vi "Scripting_OpenViRef.vi"(8 "error in":errorcluster, 10 "ViPath/ViName/Viref":variant, 11 "AppRef":refnum<vi>) -> (0 "error out":errorcluster, 2 "RefOpened(Needs to be closed)":bool, 3 "vi reference":refnum<vi>)   [LabVIEW 2020]
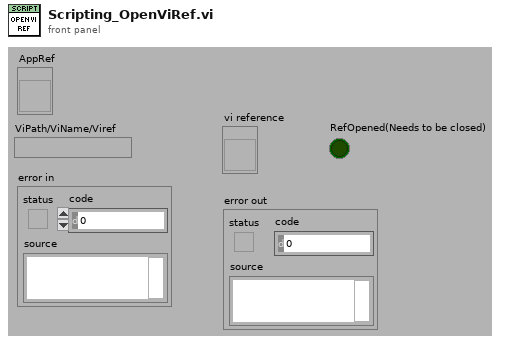
[diagram p1: front panel]
types:
  T1 = enum32{"invalid lock state", "Not Locked", "Locked (No Password)", "Password-protected"}
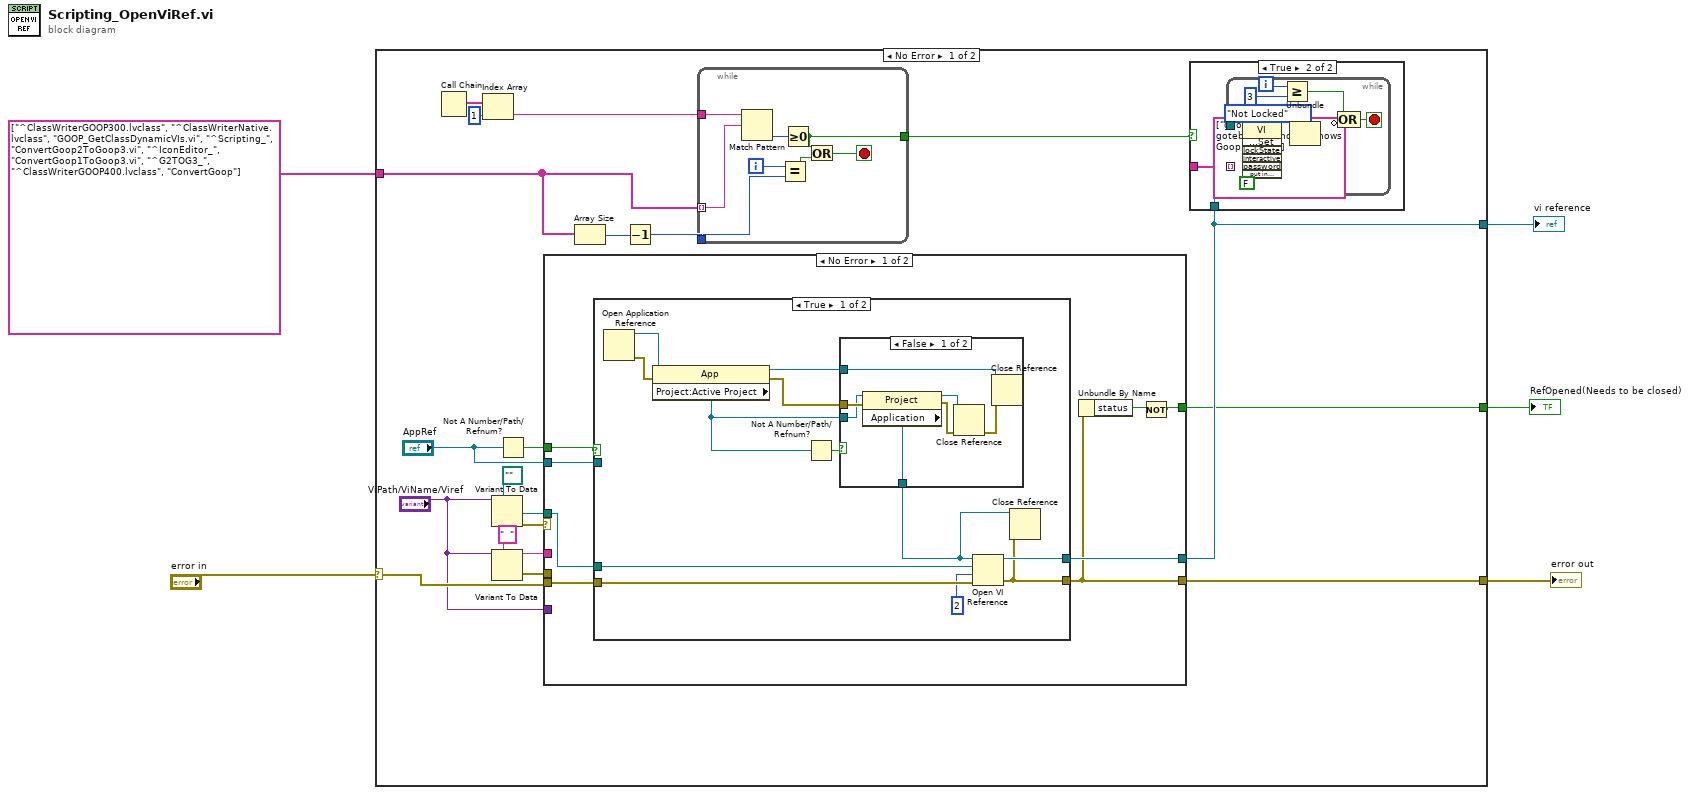
[diagram p0: block diagram]
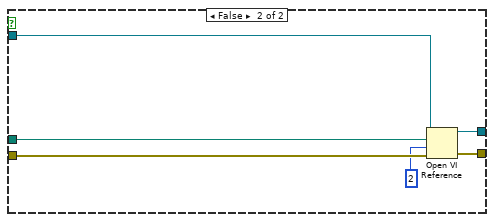
[diagram p4: hidden frame]
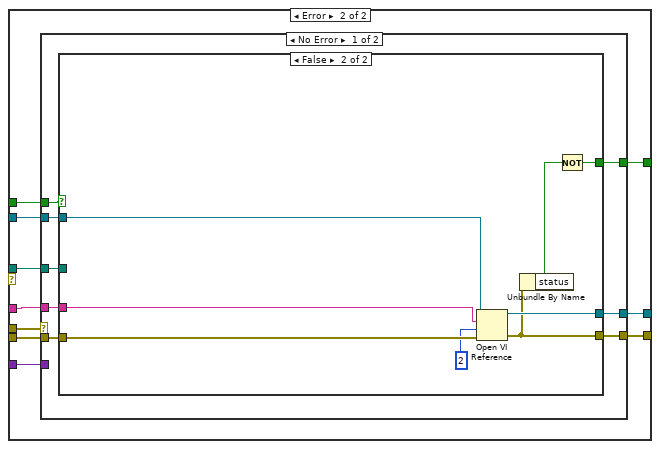
[diagram p5: hidden frame]
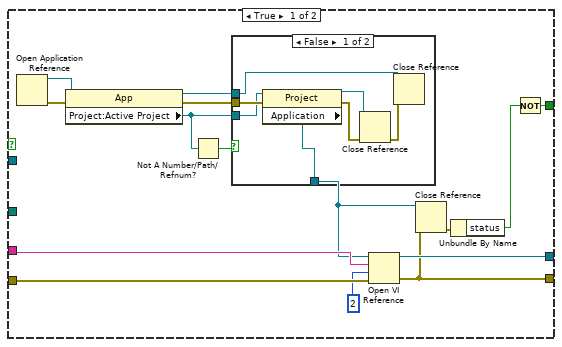
[diagram p6: hidden frame]
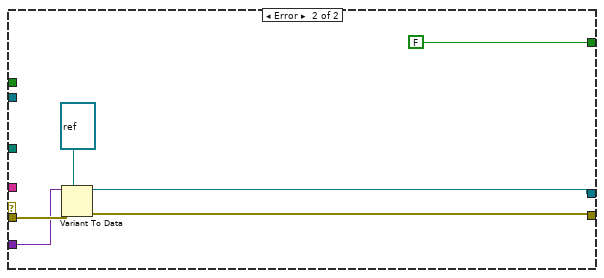
[diagram p8: hidden frame]
diagram:
  n1 = case shown="No Error" "error in" {
    selector: "error in" -> [w17 w136]
    tunnel: [w26 w136] -> w5
    tunnel: [w25 _] -> w4
    tunnel: string[] ["^ClassWriterGOOP300.lvclass", "^ClassWriterNative.lvclass", "GOOP_GetClassDynamicVIs.vi", "^Scripting_", "ConvertGoop2ToGoop3.vi", "^IconEditor_", "ConvertGoop1ToGoop3.vi", "^G2TOG3_", "^ClassWriterGOOP400.lvclass", "ConvertGoop"] -> [w9 _]
    tunnel: [w6 _] -> w1
    frame No Error {
      n2 = Call Chain() -> (call chain=w16:string[])
      n3 = Index Array(array=w16, index=1) -> (element=w14:string)
      n4 = Variant To Data(type=path "" ("vi path"), Variant="ViPath/ViName/Viref") -> (data=w23:path, error out=w22:errorcluster)  [unwired: 1 in]
      n5 = Variant To Data(type="  ", Variant="ViPath/ViName/Viref") -> (data=w18:string, error out=w8:errorcluster)  [unwired: 1 in]
      n6 = Not A Number/Path/Refnum?(number/path/refnum="AppRef") -> (NaN/Path/Refnum?=w21:bool)
      n7 = case shown="No Error" w22 {
        tunnel: w17 -> [w54 w90]
        tunnel: [w49 w89] -> w26
        tunnel: [w53 w88] -> w25
        tunnel: w23 -> [w52 w87]
        tunnel: w21 -> [w51 w86]
        tunnel: "AppRef" -> [w50 w85]
        tunnel: w18 -> [_ w84]
        tunnel: w8 -> [_ w83]
        tunnel: "ViPath/ViName/Viref" -> [_ w82]
        tunnel: [w47 w81] -> w6
        frame No Error {
          n8 = case shown="True" w51 {
            tunnel: w54 -> [w66 w80]
            tunnel: [w60 w79] -> w49
            tunnel: [w61 w78] -> w53
            tunnel: w52 -> [w64 w76]
            tunnel: w50 -> [_ w75]
            frame True {
              n9 = Open Application Reference() -> (0:w62:errorcluster, 3:w63:refnum<vi>)  [unwired: 4 in]
              n10 = property class="App"(reference=w63, error in=w62) -> (reference out=w55:refnum<vi>, error out=w56:errorcluster, "Project:Active Project"=w57:refnum<vi>)
              n11 = Not A Number/Path/Refnum?(number/path/refnum=w57) -> (NaN/Path/Refnum?=w59:bool)
              n12 = case shown="False" w59 {
                tunnel: w56 -> [w73 _]
                tunnel: [w72 w74] -> w58
                tunnel: w57 -> [w71 _]
                tunnel: w55 -> [w70 w74]
                frame False {
                  n13 = property class="Project"(reference=w71, error in=w73) -> (reference out=w67:refnum<vi>, error out=w69:errorcluster, "Application"=w72:refnum<vi>)
                  n14 = Close Reference(reference=w67, error in (no error)=w69) -> (error out=w68:errorcluster)
                  n15 = Close Reference(reference=w70, error in (no error)=w68) -> ()  [unwired: 1 out]
                }
                frame True {
                }
              }
              n16 = Open VI Reference(application reference (local)=w58, vi path=w64, options=2, error in (no error)=w66) -> (vi reference=w61:refnum<vi>, error out=w60:errorcluster)  [unwired: 2 in]
              n17 = Close Reference(reference=w58, error in (no error)=w60) -> ()  [unwired: 1 out]
            }
            frame False {
              n18 = Open VI Reference(application reference (local)=w75, vi path=w76, options=2, error in (no error)=w80) -> (vi reference=w78:refnum<vi>, error out=w79:errorcluster)  [unwired: 2 in]
            }
          }
          n19 = Unbundle By Name(w49) -> ("status"=w48:bool)
          n20 = Not(x=w48) -> (.not. x?=w47:bool)
        }
        frame Error {
          n21 = case shown="No Error" w83 {
            tunnel: w90 -> [w98 w135]
            tunnel: [w97 w132] -> w89
            tunnel: [w96 w131] -> w88
            tunnel: w87 -> [w95 _]
            tunnel: w86 -> [w94 _]
            tunnel: w85 -> [w93 _]
            tunnel: w84 -> [w92 _]
            tunnel: w82 -> [_ w134]
            tunnel: [w91 FALSE] -> w81
            frame No Error {
              n22 = case shown="False" w94 {
                tunnel: w98 -> [w113 w129]
                tunnel: [w105 w124] -> w97
                tunnel: [w112 w128] -> w96
                tunnel: w95 -> [_ _]
                tunnel: w93 -> [_ w126]
                tunnel: w92 -> [w110 w125]
                tunnel: [w99 w123] -> w91
                frame True {
                  n23 = Open Application Reference() -> (0:w106:errorcluster, 3:w107:refnum<vi>)  [unwired: 4 in]
                  n24 = property class="App"(reference=w107, error in=w106) -> (reference out=w109:refnum<vi>, error out=w108:errorcluster, "Project:Active Project"=w103:refnum<vi>)
                  n25 = Not A Number/Path/Refnum?(number/path/refnum=w103) -> (NaN/Path/Refnum?=w102:bool)
                  n26 = case shown="False" w102 {
                    tunnel: w109 -> [w120 w121]
                    tunnel: w108 -> [w119 _]
                    tunnel: [w118 w121] -> w104
                    tunnel: w103 -> [w117 _]
                    frame False {
                      n27 = property class="Project"(reference=w117, error in=w119) -> (reference out=w114:refnum<vi>, error out=w116:errorcluster, "Application"=w118:refnum<vi>)
                      n28 = Close Reference(reference=w114, error in (no error)=w116) -> (error out=w115:errorcluster)
                      n29 = Close Reference(reference=w120, error in (no error)=w115) -> ()  [unwired: 1 out]
                    }
                    frame True {
                    }
                  }
                  n30 = Open VI Reference(application reference (local)=w104, vi path=w110, options=2, error in (no error)=w113) -> (vi reference=w112:refnum<vi>, error out=w105:errorcluster)  [unwired: 2 in]
                  n31 = Close Reference(reference=w104, error in (no error)=w105) -> (error out=w101:errorcluster)
                  n32 = Unbundle By Name(w101) -> ("status"=w100:bool)
                  n33 = Not(x=w100) -> (.not. x?=w99:bool)
                }
                frame False {
                  n34 = Open VI Reference(application reference (local)=w126, vi path=w125, options=2, error in (no error)=w129) -> (vi reference=w128:refnum<vi>, error out=w124:errorcluster)  [unwired: 2 in]
                  n35 = Unbundle By Name(w124) -> ("status"=w122:bool)
                  n36 = Not(x=w122) -> (.not. x?=w123:bool)
                }
              }
            }
            frame Error {
              n37 = Variant To Data(error in=w135, type=refnum<vi> refnum ("vi reference"), Variant=w134) -> (data=w131:refnum<vi>, error out=w132:errorcluster)
            }
          }
        }
      }
      n38 = Array Size(array=w9) -> (size(s)=w12:i32)
      n39 = Decrement(x=w12) -> (x-1=w11:i32)
      n40 = while {
        tunnel: w14 -> [w46]
        tunnel: w9 -> [w45] mode=indexing
        tunnel: [w40] -> w13
        tunnel: w11 -> [w39]
        i -> [w43]
        stop <- w41 stop-if-true
        n41 = Match Pattern(string=w46, regular expression=w45) -> (offset past match=w44:i32)  [unwired: 1 in, 3 out]
        n42 = Equal?(x=w43, y=w39) -> (x = y?=w42:bool)
        n43 = Greater Or Equal To 0?(x=w44) -> (x >= 0?=w40:bool)
        n44 = Or(x=w40, y=w42) -> (x .or. y?=w41:bool)
      }
      n45 = case shown="True" w13 {
        tunnel: w25 -> [_ w28]
        tunnel: string[] ["goop rules", "i love goteborg", "Endevo Knows Goop!", "kiss"] -> [_ w27]
        frame False {
        }
        frame True {
          n46 = while {
            tunnel: w28 -> [w36]
            tunnel: w27 -> [w35] mode=indexing
            i -> [w32]
            stop <- w33 stop-if-true
            w37 = FALSE ("Interactive")
            n47 = invoke class="VI" method="Lock State.Set"(reference=w36, "lockState"=T1."Not Locked" ("Lock State"), "interactive"=w37, "password"=w35, "put in Cache"=w37) -> (error out=w34:errorcluster)  [unwired: 2 in, 6 out]
            n48 = Greater Or Equal?(x=w32, y=3) -> (x >= y?=w31:bool)
            n49 = Unbundle(w34) -> ("status"=w29:bool)  [unwired: 2 out]
            n50 = Compound Arithmetic op=OR(w31, invert w29) -> (w33:bool)
          }
        }
      }
    }
    frame Error {
    }
  }
  "vi reference" <- w4
  "error out" <- w5
  "RefOpened(Needs to be closed)" <- w1
